vi "Unload VI From Memory.vi"(8 "error in (no error)":errorcluster, 10 "VI Path":path, 11 "Session in":refnum<class "Session.lvclass">) -> (0 "error out":errorcluster, 3 "Session out":refnum<class "Session.lvclass">)   [LabVIEW 2020, in "Save for Previous Version.lvlib" / "Session.lvclass"]
uses:
  Session.lvclass
  Session.lvclass/Session.ctl
  VI File/VI File.lvclass
  <userlib>/_OpenG.lib/file/file.llb/Append Path to Root if Relative - Scalar__ogtk.vi
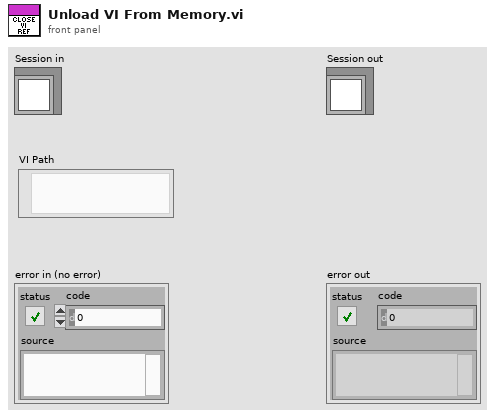
[diagram p1: front panel]
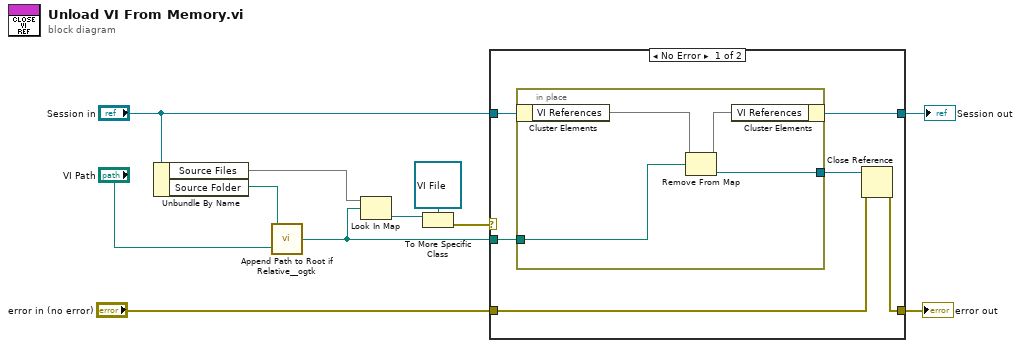
[diagram p0: block diagram]
diagram:
  n1 = Unbundle By Name("Session in") -> ("Source Files"=w7:map{path, refnum<class "File.lvclass">}, "Source Folder"=w8:path)
  n2 = call-poly <userlib>:"Append Path to Root if Relative__ogtk.vi"("Absolute or Relative Path"="VI Path", "Root Path"=w8) -> ("Absolute or Appended Path"=w1:path)
  n3 = Look In Map(map=w7, key=w1) -> (value=w5:refnum<class "File.lvclass">)  [unwired: 1 in, 1 out]
  n4 = To More Specific Class(target class=refnum<class "VI File.lvclass"> refnum ("Save for Previous Version.lvlib:VI File.lvclass"), reference=w5) -> (error out=w2:errorcluster)  [unwired: 1 in, 1 out]
  n5 = case shown="No Error" w2 {
    tunnel: [w17 w23] -> w11
    tunnel: "error in (no error)" -> [w15 w22]
    tunnel: [w14 w22] -> w9
    tunnel: "Session in" -> [w13 w23]
    tunnel: w1 -> [w12 _]
    frame No Error {
      n6 = in-place {
        in-place-border: [w19] -> w16
        in-place-border: w12 -> [w18]
        n7 = in-place-cluster #1(w13) -> ("VI References"=w21:map{path, refnum<vi>})
        n8 = Remove From Map(10:w18, 11:w21) -> (1:w19:refnum<vi>, 3:w20:map{path, refnum<vi>})  [unwired: 1 out]
        n9 = in-place-cluster #1("VI References"=w20) -> (w17:refnum<class "Session.lvclass">)
      }
      n10 = Close Reference(reference=w16, error in (no error)=w15) -> (error out=w14:errorcluster)
    }
    frame Error {
    }
  }
  "Session out" <- w11
  "error out" <- w9
